vi "Change Period.vi"(8 "error in":errorcluster, 10 "Period [ms]":i32, 11 "Helper Loop":refnum<class "Helper Loop DQMH.lvclass">) -> (0 "error out":errorcluster, 3 "Helper Loop Out":refnum<class "Helper Loop DQMH.lvclass">)   [LabVIEW 2026, in "Helper Loop DQMH.lvclass"]
doc: "周期的に送る周期を変更します。\n変更すると、それまで経過した時間がリセットされます。"
uses:
  Helper Loop DQMH.lvclass
  Helper Loop DQMH.lvclass/Helper Loop DQMH.ctl
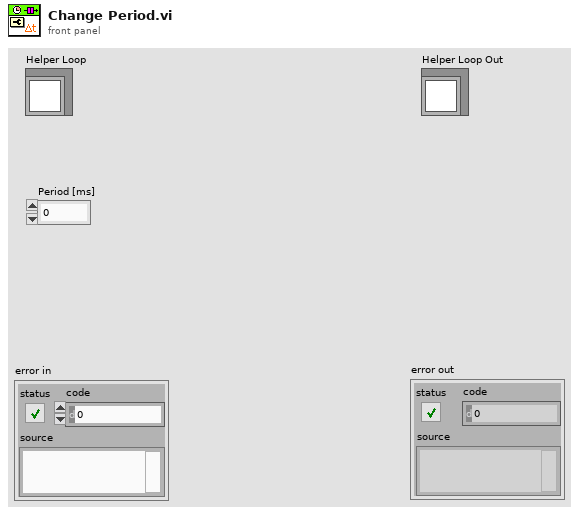
[diagram p1: front panel]
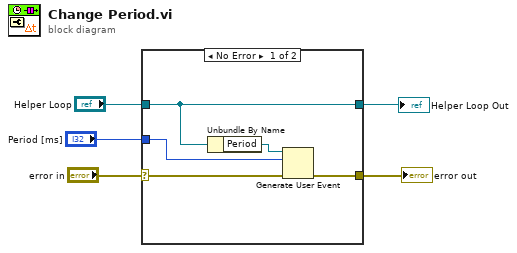
[diagram p0: block diagram]
diagram:
  n1 = case shown="No Error" "error in" {
    selector: "error in" -> [w8 w12]
    tunnel: [w7 w12] -> w4
    tunnel: "Helper Loop" -> [w10 w11]
    tunnel: [w10 w11] -> w2
    tunnel: "Period [ms]" -> [w6 _]
    frame No Error {
      n2 = Unbundle By Name(w10) -> ("Period"=w9:refnum<user-event>)
      n3 = Generate User Event(user event=w9, event data cluster=w6, error in=w8) -> (error out=w7:errorcluster)  [unwired: 1 in, 1 out]
    }
    frame Error {
    }
  }
  "error out" <- w4
  "Helper Loop Out" <- w2
